vi "test modern headers.vi"(8 "error in (no error)":errorcluster) -> (0 "error out":errorcluster, 3 "body":string)   [LabVIEW 2020, in "MCP Server tests.lvlib"]
doc: "Modern requests must carry headers that repeat the body: MCP-Protocol-Version equal to params._meta protocolVersion, Mcp-Method equal to method, and for tools/call Mcp-Name equal to params.name. A missing or different header is refused with HTTP 400 and error -32020 (header mismatch). An Mcp-Name in the form =?base64?...?= is decoded before the comparison, and header names are not case-sensitive. The requests are sent with the LabVIEW HTTP Client directly."
uses:
  MCP Server tests.lvlib
  <vilib>/addons/_JKI Toolkits/Caraya/classes/Test/Test.lvclass
  <vilib>/addons/_JKI Toolkits/Caraya/classes/Assert/Assert.lvclass
panel:
  out "lookup error":errorcluster
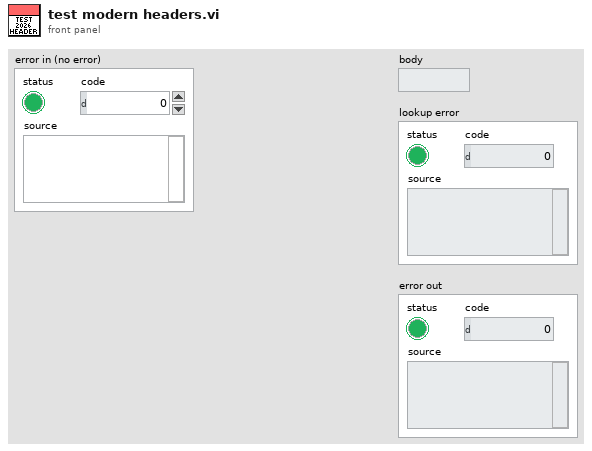
[diagram p1: front panel]
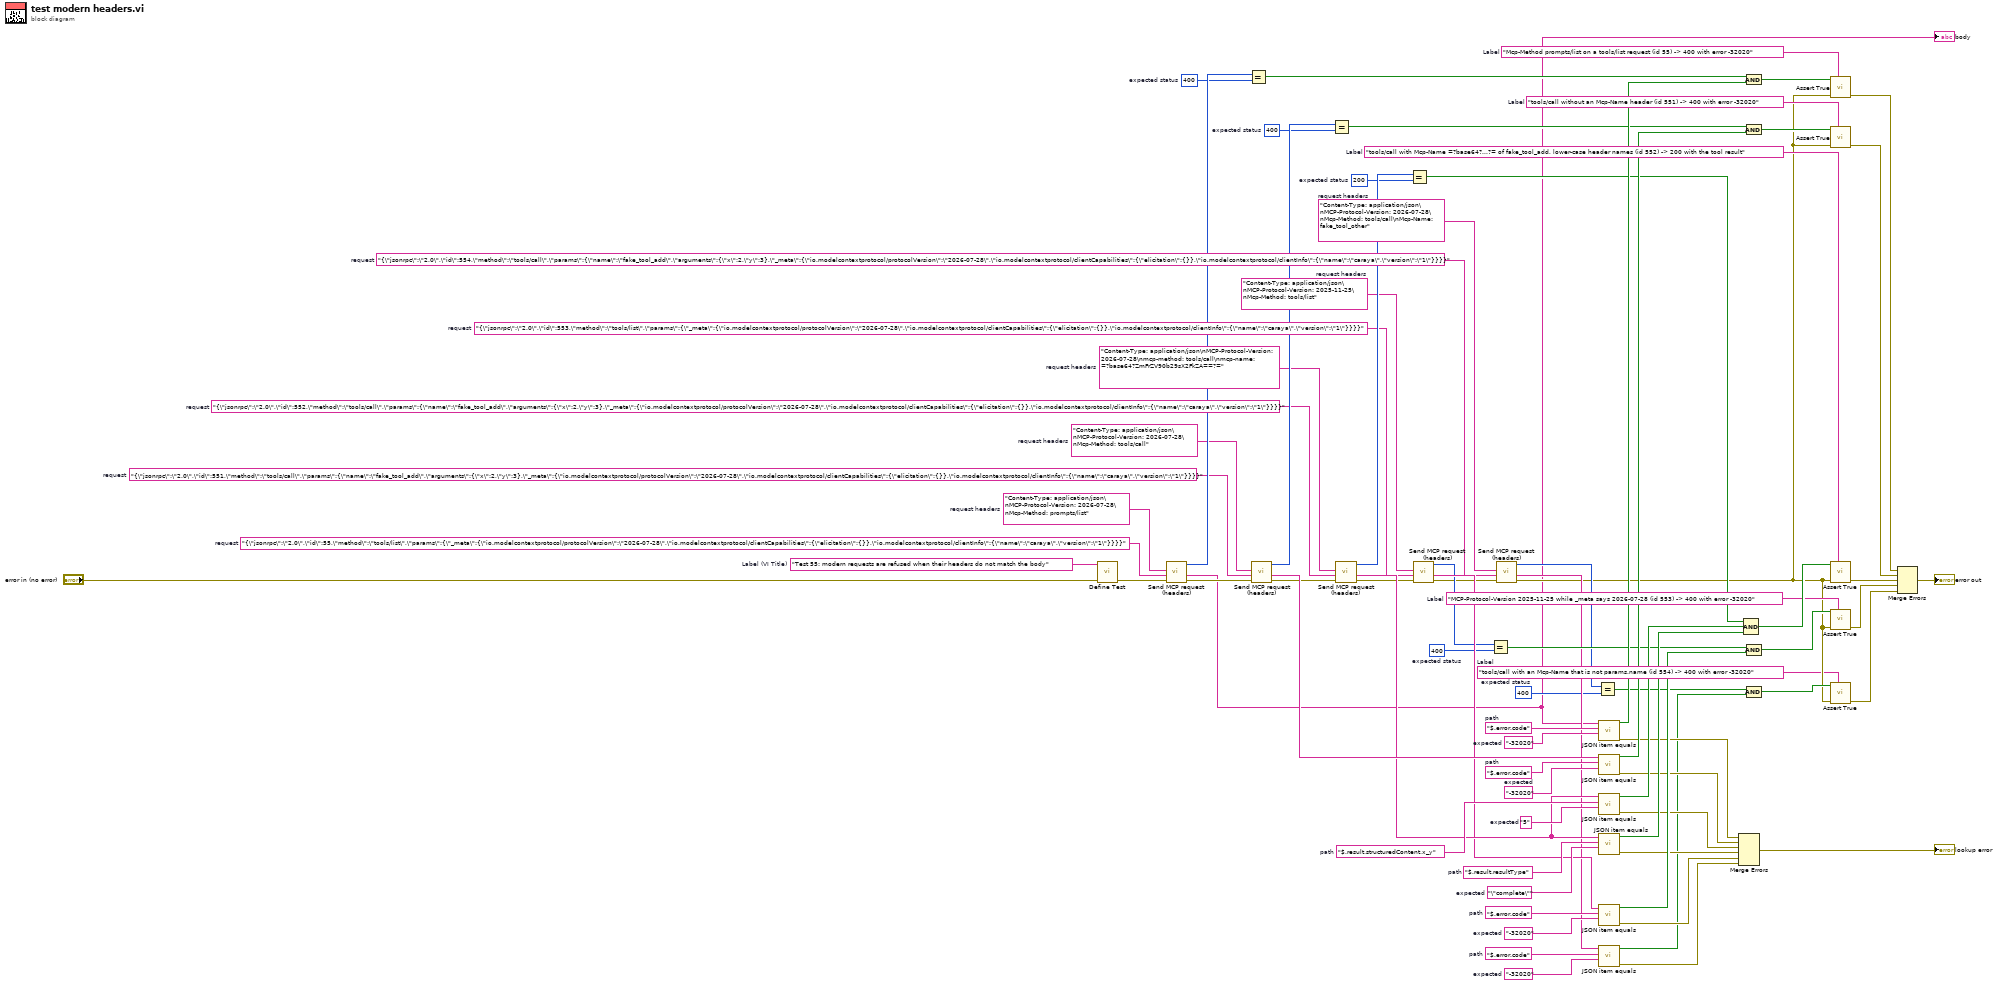
[diagram p0: block diagram]
diagram:
  w35 = "Content-Type: application/json\nMCP-Protocol-Version: 2026-07-28\nMcp-Method: tools/call\nMcp-Name: fake_tool_other"  # request headers
  w45 = "Content-Type: application/json\nMCP-Protocol-Version: 2025-11-25\nMcp-Method: tools/list"  # request headers
  w58 = "Content-Type: application/json\nMCP-Protocol-Version: 2026-07-28\nmcp-method: tools/call\nmcp-name: =?base64?ZmFrZV90b29sX2FkZA==?="  # request headers
  w68 = "Content-Type: application/json\nMCP-Protocol-Version: 2026-07-28\nMcp-Method: tools/call"  # request headers
  w77 = "Content-Type: application/json\nMCP-Protocol-Version: 2026-07-28\nMcp-Method: prompts/list"  # request headers
  w9 = "tools/call with an Mcp-Name that is not params.name (id 554) -> 400 with error -32020"  # Label
  w16 = "MCP-Protocol-Version 2025-11-25 while _meta says 2026-07-28 (id 553) -> 400 with error -32020"  # Label
  w18 = "tools/call with Mcp-Name =?base64?...?= of fake_tool_add, lower-case header names (id 552) -> 200 with the tool result"  # Label
  w20 = "tools/call without an Mcp-Name header (id 551) -> 400 with error -32020"  # Label
  w22 = "Mcp-Method prompts/list on a tools/list request (id 55) -> 400 with error -32020"  # Label
  w25 = "-32020"  # expected
  w26 = "$.error.code"  # path
  w14 = 400  # expected status
  w40 = "-32020"  # expected
  w41 = "$.error.code"  # path
  w38 = 400  # expected status
  w51 = "\"complete\""  # expected
  w52 = "$.result.resultType"  # path
  w54 = "5"  # expected
  w55 = "$.result.structuredContent.x_y"  # path
  w49 = 200  # expected status
  w63 = "-32020"  # expected
  w64 = "$.error.code"  # path
  w61 = 400  # expected status
  w73 = "-32020"  # expected
  w74 = "$.error.code"  # path
  w71 = 400  # expected status
  w34 = "{\"jsonrpc\":\"2.0\",\"id\":554,\"method\":\"tools/call\",\"params\":{\"name\":\"fake_tool_add\",\"arguments\":{\"x\":2,\"y\":3},\"_meta\":{\"io.modelcontextprotocol/protocolVersion\":\"2026-07-28\",\"io.modelcontextprotocol/clientCapabilities\":{\"elicitation\":{}},\"io.modelcontextprotocol/clientInfo\":{\"name\":\"caraya\",\"version\":\"1\"}}}}"  # request
  w44 = "{\"jsonrpc\":\"2.0\",\"id\":553,\"method\":\"tools/list\",\"params\":{\"_meta\":{\"io.modelcontextprotocol/protocolVersion\":\"2026-07-28\",\"io.modelcontextprotocol/clientCapabilities\":{\"elicitation\":{}},\"io.modelcontextprotocol/clientInfo\":{\"name\":\"caraya\",\"version\":\"1\"}}}}"  # request
  w57 = "{\"jsonrpc\":\"2.0\",\"id\":552,\"method\":\"tools/call\",\"params\":{\"name\":\"fake_tool_add\",\"arguments\":{\"x\":2,\"y\":3},\"_meta\":{\"io.modelcontextprotocol/protocolVersion\":\"2026-07-28\",\"io.modelcontextprotocol/clientCapabilities\":{\"elicitation\":{}},\"io.modelcontextprotocol/clientInfo\":{\"name\":\"caraya\",\"version\":\"1\"}}}}"  # request
  w67 = "{\"jsonrpc\":\"2.0\",\"id\":551,\"method\":\"tools/call\",\"params\":{\"name\":\"fake_tool_add\",\"arguments\":{\"x\":2,\"y\":3},\"_meta\":{\"io.modelcontextprotocol/protocolVersion\":\"2026-07-28\",\"io.modelcontextprotocol/clientCapabilities\":{\"elicitation\":{}},\"io.modelcontextprotocol/clientInfo\":{\"name\":\"caraya\",\"version\":\"1\"}}}}"  # request
  w76 = "{\"jsonrpc\":\"2.0\",\"id\":55,\"method\":\"tools/list\",\"params\":{\"_meta\":{\"io.modelcontextprotocol/protocolVersion\":\"2026-07-28\",\"io.modelcontextprotocol/clientCapabilities\":{\"elicitation\":{}},\"io.modelcontextprotocol/clientInfo\":{\"name\":\"caraya\",\"version\":\"1\"}}}}"  # request
  w79 = "Test 55: modern requests are refused when their headers do not match the body"  # Label (VI Title)
  n1 = call <vilib>:"Define Test.vi"("error in (no error)"="error in (no error)", "Label (VI Title)"=w79) -> ("error out"=w75:errorcluster)  [unwired: 8 in, 1 out]
  n2 = call "Send MCP request (headers).vi"("error in (no error)"=w75, "request"=w76, "request headers"=w77) -> ("error out"=w66:errorcluster, "response"=w3:string, "status code"=w72:i32)  [unwired: 5 in, 1 out]
  "body" <- w3
  n3 = Equal?(x=w72, y=w71) -> (x = y?=w70:bool)
  n4 = call "Send MCP request (headers).vi"("error in (no error)"=w66, "request"=w67, "request headers"=w68) -> ("error out"=w56:errorcluster, "response"=w65:string, "status code"=w62:i32)  [unwired: 5 in, 1 out]
  n5 = Equal?(x=w62, y=w61) -> (x = y?=w60:bool)
  n6 = call "Send MCP request (headers).vi"("error in (no error)"=w56, "request"=w57, "request headers"=w58) -> ("error out"=w43:errorcluster, "response"=w53:string, "status code"=w50:i32)  [unwired: 5 in, 1 out]
  n7 = Equal?(x=w50, y=w49) -> (x = y?=w48:bool)
  n8 = call "Send MCP request (headers).vi"("error in (no error)"=w43, "request"=w44, "request headers"=w45) -> ("error out"=w33:errorcluster, "response"=w42:string, "status code"=w39:i32)  [unwired: 5 in, 1 out]
  n9 = Equal?(x=w39, y=w38) -> (x = y?=w37:bool)
  n10 = call "Send MCP request (headers).vi"("error in (no error)"=w33, "request"=w34, "request headers"=w35) -> ("error out"=w10:errorcluster, "response"=w27:string, "status code"=w15:i32)  [unwired: 5 in, 1 out]
  n11 = Equal?(x=w15, y=w14) -> (x = y?=w13:bool)
  n12 = call "JSON item equals.vi"("expected"=w73, "path"=w74, "JSON"=w3) -> ("error out"=w32:errorcluster, "equal?"=w69:bool)  [unwired: 6 in, 1 out]
  n13 = call "JSON item equals.vi"("expected"=w63, "path"=w64, "JSON"=w65) -> ("error out"=w31:errorcluster, "equal?"=w59:bool)  [unwired: 6 in, 1 out]
  n14 = call "JSON item equals.vi"("expected"=w54, "path"=w55, "JSON"=w53) -> ("error out"=w30:errorcluster, "equal?"=w47:bool)  [unwired: 6 in, 1 out]
  n15 = call "JSON item equals.vi"("expected"=w51, "path"=w52, "JSON"=w53) -> ("error out"=w29:errorcluster, "equal?"=w46:bool)  [unwired: 6 in, 1 out]
  n16 = call "JSON item equals.vi"("expected"=w40, "path"=w41, "JSON"=w42) -> ("error out"=w28:errorcluster, "equal?"=w36:bool)  [unwired: 6 in, 1 out]
  n17 = call "JSON item equals.vi"("expected"=w25, "path"=w26, "JSON"=w27) -> ("error out"=w24:errorcluster, "equal?"=w12:bool)  [unwired: 6 in, 1 out]
  n18 = Merge Errors(w32, w31, w30, w29, w28, w24) -> (→"lookup error":errorcluster)
  n19 = Compound Arithmetic op=AND(w48, w47, w46) -> (w19:bool)
  n20 = Compound Arithmetic op=AND(w70, w69) -> (w23:bool)
  n21 = Compound Arithmetic op=AND(w60, w59) -> (w21:bool)
  n22 = Compound Arithmetic op=AND(w37, w36) -> (w17:bool)
  n23 = Compound Arithmetic op=AND(w13, w12) -> (w11:bool)
  n24 = call <vilib>:"Assert True.vi"("Label"=w22, "error in (no error)"=w10, "True?"=w23) -> ("error out"=w8:errorcluster)  [unwired: 7 in, 1 out]
  n25 = call <vilib>:"Assert True.vi"("Label"=w20, "error in (no error)"=w10, "True?"=w21) -> ("error out"=w7:errorcluster)  [unwired: 7 in, 1 out]
  n26 = call <vilib>:"Assert True.vi"("Label"=w18, "error in (no error)"=w10, "True?"=w19) -> ("error out"=w6:errorcluster)  [unwired: 7 in, 1 out]
  n27 = call <vilib>:"Assert True.vi"("Label"=w16, "error in (no error)"=w10, "True?"=w17) -> ("error out"=w5:errorcluster)  [unwired: 7 in, 1 out]
  n28 = call <vilib>:"Assert True.vi"("Label"=w9, "error in (no error)"=w10, "True?"=w11) -> ("error out"=w4:errorcluster)  [unwired: 7 in, 1 out]
  n29 = Merge Errors(w8, w7, w6, w5, w4) -> (→"error out":errorcluster)
